vi "Run VI.vi"(4 "MaxBuildVer":string, 6 "Buildlog":path, 8 "error in (no error)":errorcluster, 11 "VI Path":path) -> (0 "error out":errorcluster)   [LabVIEW 2011]
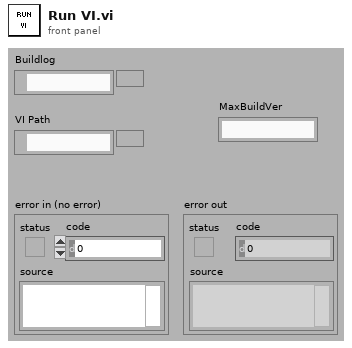
[diagram p1: front panel]
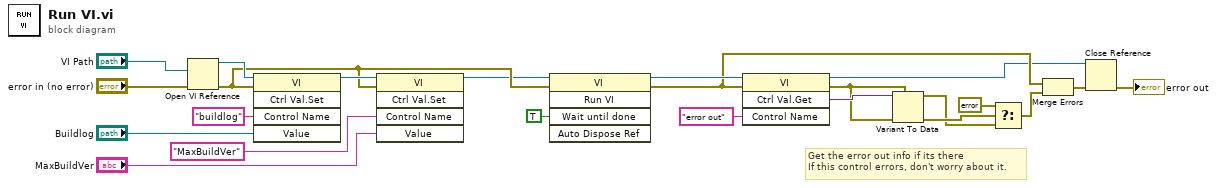
[diagram p0: block diagram]
diagram:
  # "Get the error out info if its there\nIf this control errors, don't worry about it."
  n1 = Open VI Reference(vi path="VI Path", error in (no error)="error in (no error)") -> (vi reference=w7:refnum<vi>, error out=w2:errorcluster)  [unwired: 4 in]
  n2 = invoke class="VI" method="Ctrl Val.Set"(reference=w7, error in=w2, "Control Name"="buildlog", "Value"="Buildlog") -> (reference out=w5:refnum<vi>)  [unwired: 1 in, 4 out]
  n3 = invoke class="VI" method="Ctrl Val.Set"(reference=w5, error in=w2, "Control Name"="MaxBuildVer", "Value"="MaxBuildVer") -> (reference out=w1:refnum<vi>)  [unwired: 1 in, 4 out]
  n4 = invoke class="VI" method="Run VI"(reference=w1, error in=w2, "Wait until done"=TRUE ("Wait Until Done")) -> (reference out=w20:refnum<vi>, error out=w13:errorcluster)  [unwired: 2 in, 3 out]
  n5 = invoke class="VI" method="Ctrl Val.Get"(reference=w20, error in=w13, "Control Name"="error out") -> (reference out=w9:refnum<vi>, error out=w17:errorcluster, "Get Control Value Variant"=w18:variant)  [unwired: 1 in, 1 out]
  n6 = Variant To Data(error in=w17, type=w17, Variant=w18) -> (data=w14:errorcluster, error out=w16:errorcluster)
  n7 = Select(t=errorcluster {"status"=FALSE, "code"=0, "source"=""}, s=w16, f=w14) -> (s? t:f=w12:errorcluster)
  n8 = Merge Errors(w13, w12) -> (w11:errorcluster)
  n9 = Close Reference(reference=w9, error in (no error)=w11) -> (error out=→"error out":errorcluster)
